vi "SelectByLabel.vi"(8 "error in (no error)":errorcluster, 10 "String":string, 11 "References":refnum<vi>[](array[refnum])) -> (0 "error out":errorcluster, 3 "GObject out":refnum<vi>)   [LabVIEW 2020]
panel:
  out "Array":string[](array[string])
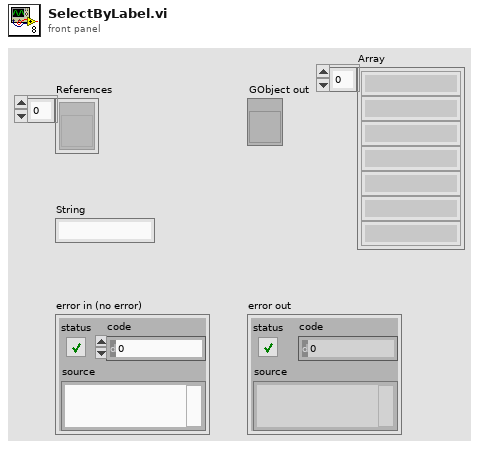
[diagram p1: front panel]
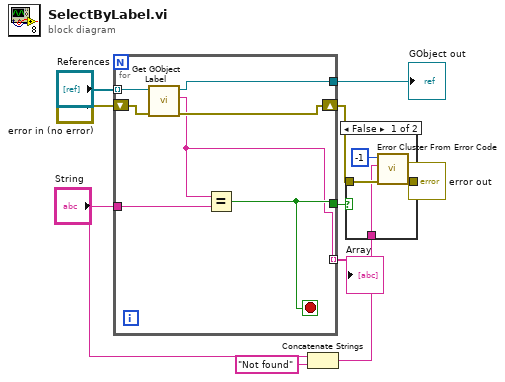
[diagram p0: block diagram]
diagram:
  n1 = for {
    tunnel: "References" -> [w17] mode=indexing
    shift-right: [w14] -> w5
    shift-left: "error in (no error)" -> [w16]
    tunnel: "String" -> [w15]
    tunnel: [w13] -> w3
    tunnel: [w12] -> w7
    tunnel: [w11] -> w1 mode=indexing
    stop <- w12 stop-if-true
    n2 = call <vilib>:"Get GObject Label.vi"("error in (no error)"=w16, "GObject"=w17) -> ("error out"=w14:errorcluster, "Object Label"=w11:string, "dup GObject"=w13:refnum<vi>)  [unwired: 5 in, 2 out]
    n3 = Equal?(x=w11, y=w15) -> (x = y?=w12:bool)
  }
  "GObject out" <- w3
  "Array" <- w1
  n4 = Concatenate Strings("String", "Not found" ("string")) -> (w9:string)
  n5 = case shown="False" w7 {
    tunnel: w5 -> [w21 w22]
    tunnel: [w20 w22] -> w6
    tunnel: w9 -> [w18 _]
    frame False {
      n6 = call <vilib>:"Error Cluster From Error Code.vi"("error in (no error)"=w21, "error message (\"\")"=w18, "error code (0)"=-1) -> ("error out"=w20:errorcluster)  [unwired: 6 in]
    }
    frame True {
    }
  }
  "error out" <- w6
